vi "variant to string.vi"(1 "Variant":variant) -> (0 "String":string)   [LabVIEW 2025]
doc: "convert variant data to a LabVIEW String\n<B>Input:</B>\nVariant (skalar)\n<B>Output:</B>\nString"
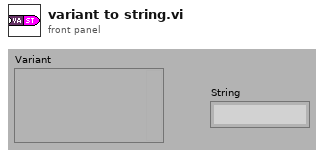
[diagram p1: front panel]
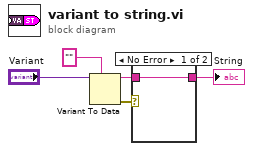
[diagram p0: block diagram]
diagram:
  n1 = Variant To Data(type="" ("MIN U/36V"), Variant="Variant") -> (data=w2:string, error out=w1:errorcluster)  [unwired: 1 in]
  n2 = case shown="No Error" w1 {
    tunnel: w2 -> [w6 _]
    tunnel: [w6 _] -> w5
    frame No Error {
    }
    frame Error {
    }
  }
  "String" <- w5
